vi "Acquerir valeur courante MODBUS.vi"(2 "Adresse régulateur":u8, 3 "Port COM run 1 REG":refnum<visa-resource-name> caption="Port RS232") -> (0 "sortie d'erreur":errorcluster, 1 "Température":dbl)   [LabVIEW 2022 SP3]
uses:
  Variables globales/Variables glob EUROTHERM.vi
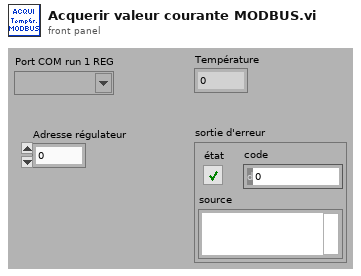
[diagram p1: front panel]
types:
  T1 = typedef "Semaphore RefNum" = refnum<k1>
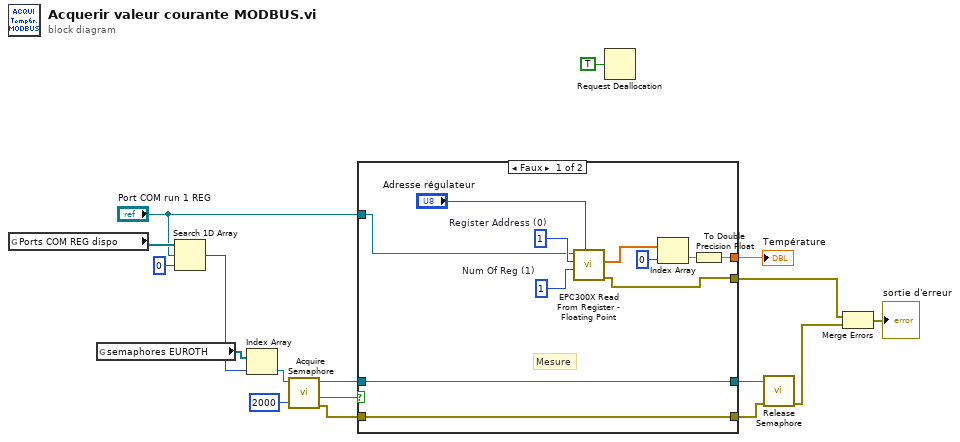
[diagram p0: block diagram]
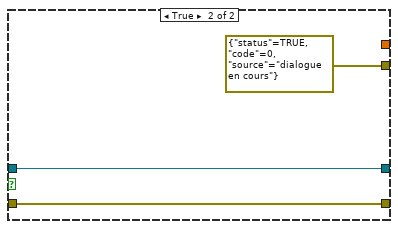
[diagram p2: hidden frame]
diagram:
  n1 = global read "Variables glob EUROTHERM.vi" "Ports COM REG dispo"() -> (w5:refnum<visa-resource-name>[])
  n2 = global read "Variables glob EUROTHERM.vi" "semaphores EUROTH"() -> (w7:T1[])
  n3 = Search 1D Array(1D array=w5, element="Port COM run 1 REG", start index (0)=0 ("indice de départ (0)")) -> (index of element=w2:i32)
  n4 = Index Array(array=w7, index=w2) -> (element=w6:T1)
  n5 = call <vilib>:"Acquire Semaphore.vi"("ms timeout (-1)"=2000, "semaphore"=w6) -> ("error out"=w13:errorcluster, "timed out"=w15:bool, "semaphore out"=w14:T1)  [unwired: 3 in]
  n6 = case shown="Faux" w15 {
    tunnel: w14 -> [w28 w31]
    tunnel: w13 -> [w27 w30]
    tunnel: [w28 w31] -> w12
    tunnel: [w27 w30] -> w11
    tunnel: [w18 errorcluster {"status"=TRUE, "code"=0, "source"="dialogue en cours"} ("error out")] -> w10
    tunnel: "Port COM run 1 REG" -> [w22 _]
    tunnel: [w26 _] -> w1
    frame False {
      w25 = u16 1  # Register Address (0)
      w24 = u16 1  # Num Of Reg (1)
      # "Mesure"
      n7 = call "EPC300X Read From Register - Floating Point.vi"("Unit Address (1)"="Adresse régulateur", "Num Of Reg (1)"=w24, "Register Address (0)"=w25, "VISA session"=w22) -> ("error out"=w18:errorcluster, "Data (SGL)"=w21:sgl[])  [unwired: 2 in, 4 out]
      n8 = Index Array(array=w21, index=0 ("indice")) -> (element=w19:sgl)
      n9 = To Double Precision Float(number=w19) -> (double precision float=w26:dbl)
    }
    frame True {
    }
  }
  "Température" <- w1
  n10 = Request Deallocation(TRUE ("flag")) -> ()
  n11 = call <vilib>:"Release Semaphore.vi"("error in (no error)"=w11, "semaphore"=w12) -> ("error out"=w9:errorcluster)  [unwired: 4 in, 1 out]
  n12 = Merge Errors(w10, w9) -> (→"sortie d'erreur":errorcluster)
